vi "Compare VS Config to Database Changes.vi"(8 "error in (no error)":errorcluster, 9 "VS Existing Frames":T10 {"Incoming"."Node Ref" format="%.0x"; "Outgoing"."Node Ref" format="%.0x"}, 10 "Old Cluster":refnum<k21>, 11 "New Cluster":refnum<k21>) -> (0 "error out":errorcluster, 3 "VS Filtered Change List":T1 {"Incoming"."Missing"."Node Ref" format="%.0x"; "Incoming"."Changed"."Old"."Node Ref" format="%.0x"; "Outgoing"."Missing"."Node Ref" format="%.0x"; "Outgoing"."Changed"."Old"."Node Ref" format="%.0x"})   [LabVIEW 2025, in "Protection and Counter Addon System Explorer.lvlib"]
uses:
  Protection and Counter Addon System Explorer.lvlib
  Types/Database Changes VS Existing Frames.ctl
  Types/Base Frame Info.ctl
  <vilib>/NI VeriStand/Custom Device API/Custom Device Item Ref.ctl
  Types/CAN Filter Type.ctl
  Types/Filtered XNET Changes.ctl
  Types/Database Changes.ctl
  Types/Base Frame Info_NoVS.ctl
  Types/Signal Attributes.ctl
  Types/Related CAN Frames.ctl
  Types/Related CAN Frames No VS.ctl
  <vilib>/NI VeriStand/Custom Device API/Custom Device API.lvlib
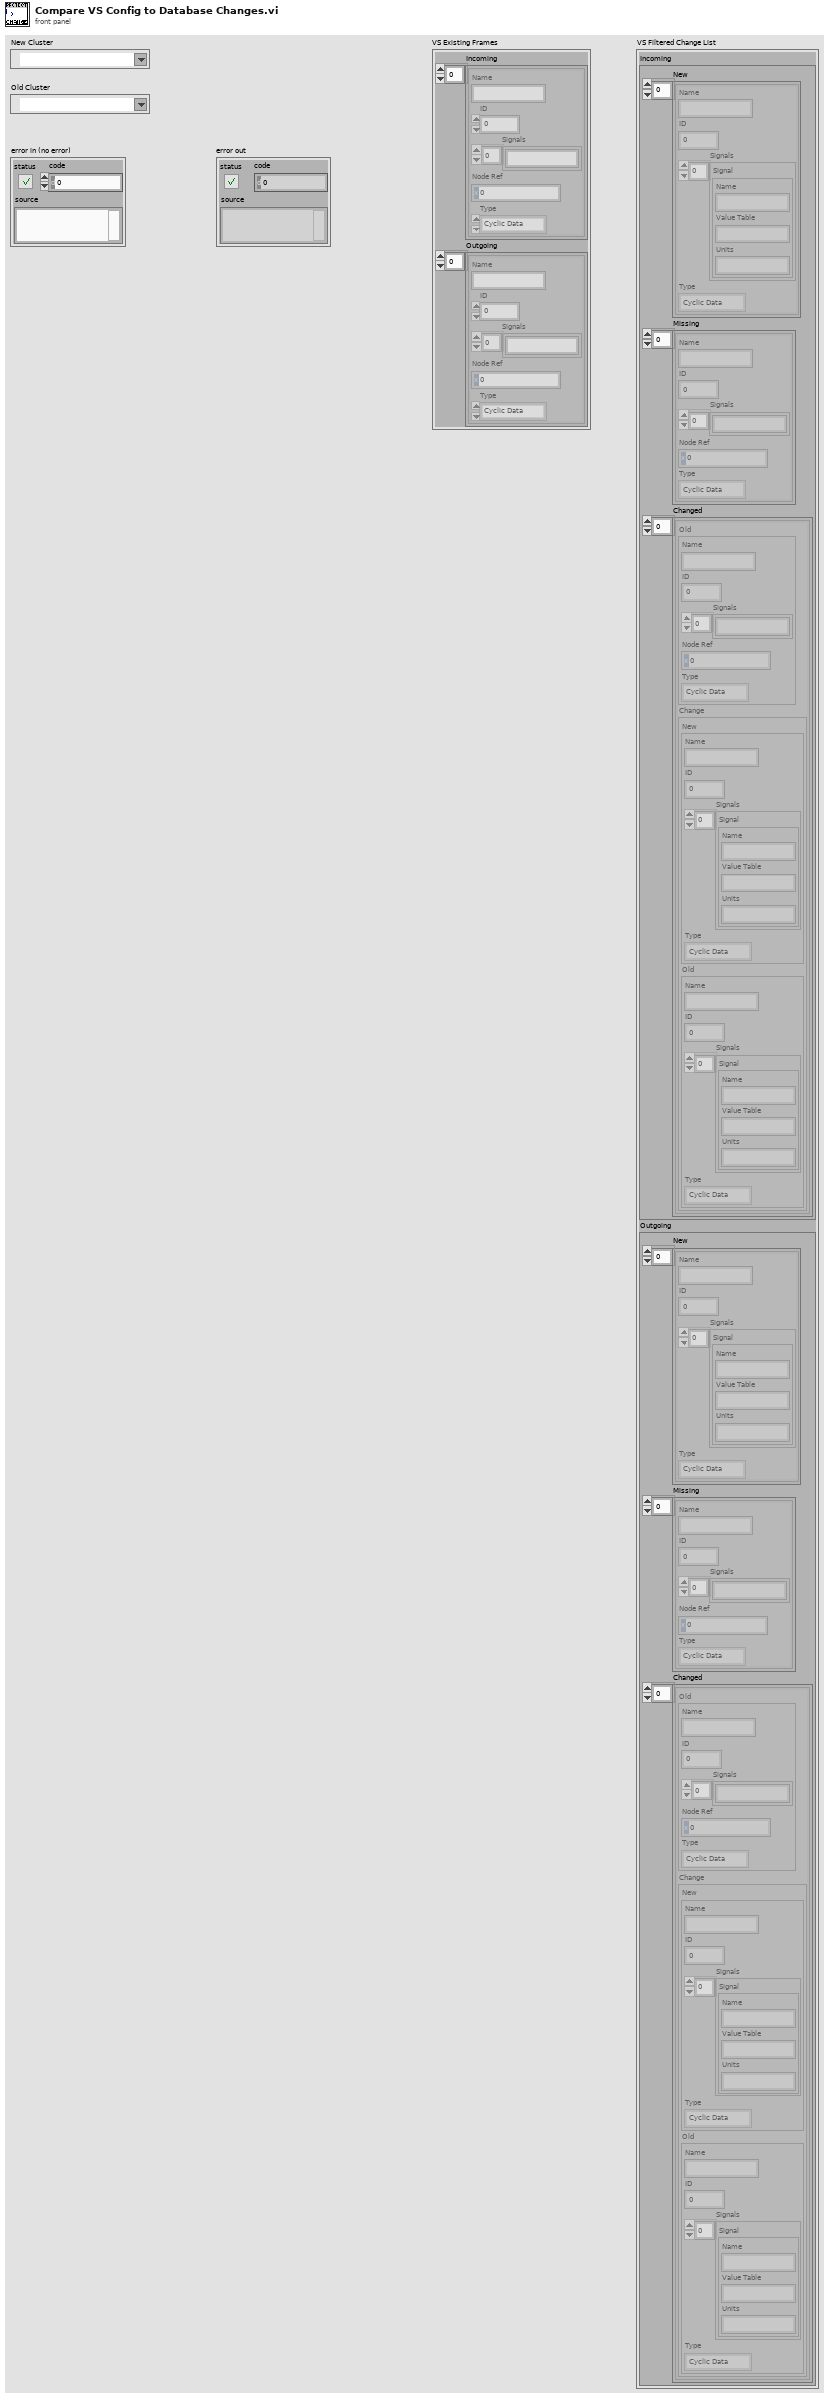
[diagram p1: front panel]
types:
  T1 = typedef "Protection and Counter Addon System Explorer.lvlib/Filtered XNET Changes.ctl" = cluster{"Incoming":T2, "Outgoing":T2}
  T2 = typedef "Protection and Counter Addon System Explorer.lvlib/Database Changes.ctl" = cluster{"New":T3[], "Missing":T6[], "Changed":T8[]}
  T3 = typedef "Protection and Counter Addon System Explorer.lvlib/Base Frame Info_NoVS.ctl" = cluster{"Name":string, "ID":u32, "Signals":T4[], "Type":T5}
  T4 = typedef "Protection and Counter Addon System Explorer.lvlib/Signal Attributes.ctl" = cluster{"Name":string, "Value Table":string, "Units":string}
  T5 = typedef "Protection and Counter Addon System Explorer.lvlib/CAN Filter Type.ctl" = enum16{"Cyclic Data", "Event Data", "Cyclic/Event", "All"}
  T6 = typedef "Protection and Counter Addon System Explorer.lvlib/Base Frame Info.ctl" = cluster{"Name":string, "ID":u32, "Signals":string[], "Node Ref":T7, "Type":T5}
  T7 = typedef "Custom Device API.lvlib/Custom Device Item Ref.ctl" = u64
  T8 = typedef "Protection and Counter Addon System Explorer.lvlib/Related CAN Frames.ctl" = cluster{"Old":T6, "Change":T9}
  T9 = typedef "Protection and Counter Addon System Explorer.lvlib/Related CAN Frames No VS.ctl" = cluster{"New":T3, "Old":T3}
  T10 = typedef "Protection and Counter Addon System Explorer.lvlib/Database Changes VS Existing Frames.ctl" = cluster{"Incoming":T6[], "Outgoing":T6[]}
  T11 = typedef "Protection and Counter Addon System Explorer.lvlib/XNET Change List.ctl" = cluster{"New":T3[], "Missing":T3[], "Changed":T9[]}
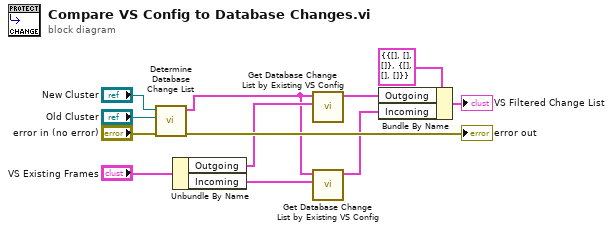
[diagram p0: block diagram]
diagram:
  n1 = call "Determine Database Change List.vi"("error in (no error)"="error in (no error)", "Old Cluster"="Old Cluster", "New Cluster"="New Cluster") -> ("error out"=→"error out":errorcluster, "XNET Change List"=w5:T11)  [unwired: 7 in]
  n2 = Unbundle By Name("VS Existing Frames") -> ("Outgoing"=w7:T6[], "Incoming"=w6:T6[])
  n3 = call "Get Database Change List by Existing VS Config.vi"("VS Existing Frames"=w7, "XNET Change List"=w5) -> ("Filtered VS Change List"=w4:T2)  [unwired: 9 in]
  n4 = call "Get Database Change List by Existing VS Config.vi"("VS Existing Frames"=w6, "XNET Change List"=w5) -> ("Filtered VS Change List"=w2:T2)  [unwired: 9 in]
  n5 = Bundle By Name(cluster=T1 {"Incoming"={"New"=[], "Missing"=[], "Changed"=[]}, "Outgoing"={"New"=[], "Missing"=[], "Changed"=[]}}, "Outgoing"=w4, "Incoming"=w2) -> (→"VS Filtered Change List":T1)
